vi "Client Monitor.vi"() -> ()   [LabVIEW 2020]
uses:
  source/Client/Client/Client.lvclass
  source/Client/Subscription/Subscription.lvclass
  source/Client/Subscription/Next Value - DBL.vi
panel:
  in  "PV name":string="DEV:FLOAT64"
  out "Timestamp":timestamp
  out "Value":dbl
  out "timed out?":bool
  in  "stop":bool
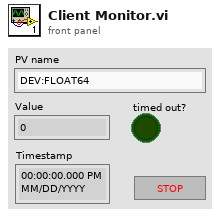
[diagram p1: front panel]
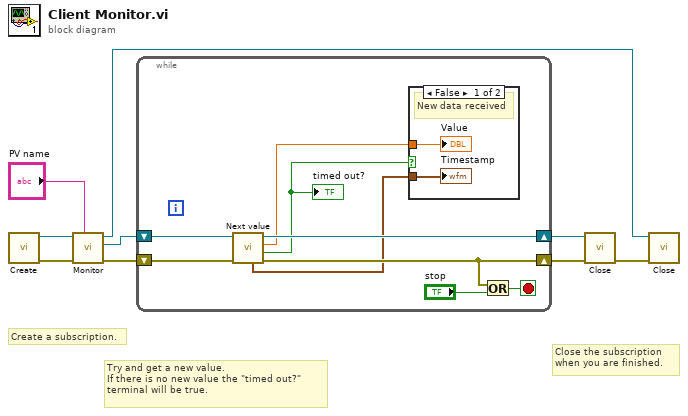
[diagram p0: block diagram]
diagram:
  # "Close the subscription when you are finished."
  # "Try and get a new value.\nIf there is no new value the \"timed out?\" terminal will be true."
  # "Create a subscription."
  n1 = call "Create.vi"() -> ("error out"=w8:errorcluster, "Client out"=w9:refnum<class "Client.lvclass">)  [unwired: 10 in]
  n2 = call "Monitor.vi"("PV name"="PV name", "error in"=w8, "Client in"=w9) -> ("error out"=w7:errorcluster, "subscription"=w5:refnum<class "Subscription.lvclass">, "Client out"=w1:refnum<class "Client.lvclass">)  [unwired: 6 in]
  n3 = while {
    shift-right: [w15] -> w3
    shift-left: w7 -> [w16]
    shift-right: [w13] -> w4
    shift-left: w5 -> [w14]
    stop <- w18 stop-if-true
    n4 = call-poly "Next value.vi"("error in (no error)"=w16, "Subscription in"=w14) -> ("error out"=w15:errorcluster, "timed out?"=w12:bool, "value"=w11:dbl, "Subscription out"=w13:refnum<class "Subscription.lvclass">, "timestamp"=w10:timestamp)  [unwired: 4 in, 1 out]
    "timed out?" <- w12
    n5 = case shown="False" w12 {
      tunnel: w11 -> [w20 _]
      tunnel: w10 -> [w19 _]
      frame False {
        # "New data received"
        "Value" <- w20
        "Timestamp" <- w19
      }
      frame True {
      }
    }
    n6 = Or(x=w15, y="stop") -> (x .or. y?=w18:bool)
  }
  n7 = call-dynamic "Close.vi"("error in (no error)"=w3, "Subscription in"=w4) -> ("error out"=w2:errorcluster)  [unwired: 9 in]
  n8 = call "Close.vi"("error in (no error)"=w2, "Client in"=w1) -> ()  [unwired: 9 in, 1 out]
